vi "MQTT Session - Get TCP Info.vi"(0 "mqtt ref in":T1, 11 "error in":errorcluster) -> (4 "mqtt ref out":T1, 6 "TCP ref":refnum<k5>, 8 "TCP Timeout (ms)":i32, 10 "Version":u8, 15 "error out":errorcluster)   [LabVIEW 2019, in "KoRE-MQTT.lvlib"]
doc: "Copyright (c) 2025 KoRElibs.com\nSPDX-License-Identifier: EUPL-1.2\n\nThis VI is licensed under the European Union Public License (EUPL) Version 1.2. You may use this VI unmodified in proprietary works. If you distribute a modified version of this file, the modified file must be released under the EUPL-1.2. Full license: https://joinup.ec.europa.eu/asset/eupl/eupl/1.2/"
uses:
  KoRE-MQTT.lvlib
  Public/TypeDefs/MQTT Client Session.ctl
  TypeDefs/MQTT Client Session - Data Value Reference.ctl
  Public/TypeDefs/MQTT Client Session - Data.ctl
  Public/TypeDefs/MQTT Property - Will.ctl
  Public/TypeDefs/MQTT Property - CONNECT.ctl
  TypeDefs/MQTT Subscription - Info.ctl
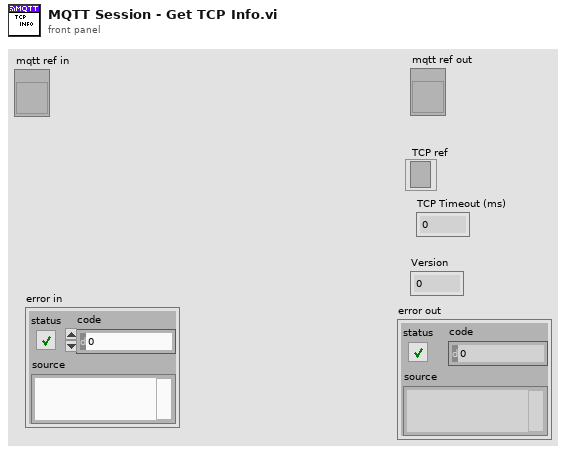
[diagram p1: front panel]
types:
  T1 = typedef "KoRE-MQTT.lvlib/MQTT Client Session.ctl" = refnum<vi>
  T2 = typedef "KoRE-MQTT.lvlib/MQTT Client Session - Data Value Reference.ctl" = refnum<data-value>
  T3 = typedef "KoRE-MQTT.lvlib/MQTT Client Session - Data.ctl" = cluster{"TCP ref":refnum<k5>, "Next Packet Id":u16, "Version":u8, "Host":string, "Port":u16, "Ping Delta":u32, "Username":string, "Password":string, "Will QoS":u8, "Will Retain":bool, "Will Topic":string, "Will Payload":string, "TCP Timeout":i32, "Semaphore":T4, "In-Flight Messages":variant, "Close":bool, "Last Send":u32, "Keep Alive":u16, "Last Ping RTT":u32, "Last Ping":u32, "Will Properties":T5[], "Session Expiry Interval":u32, "Maximum QoS":u8, "Retain Available":bool, "Server Maximum Packet Size":u32, "Client Identifier":string, "Server Topic Alias Maximum":u16, "Wildcard Subscription Available":bool, "Subscription Identifier Available":bool, "Shared Subscription Available":bool, "Connect Properties":T6[], "Client Maximum Packet Size":u32, "Client Topic Alias Maximum":u16, "Server Receive Maximum":u16, "Client Receive Maximum":u16, "TLS cfg":refnum<k36>, "Subscriptions":T7[]}
  T4 = typedef "Semaphore RefNum" = refnum<k1>
  T5 = typedef "KoRE-MQTT.lvlib/MQTT Property - Will.ctl" = cluster{"Property":u8, "Value":string}
  T6 = typedef "KoRE-MQTT.lvlib/MQTT Property - CONNECT.ctl" = cluster{"Property":u8, "Value":string}
  T7 = typedef "KoRE-MQTT.lvlib/MQTT Subscription - Info.ctl" = cluster{"Packet Id":u16, "Index":u16, "Identifier":u32, "QoS":u8, "Topic Filter":string, "Reason Code":u8, "Reason String":string, "Granted":bool}
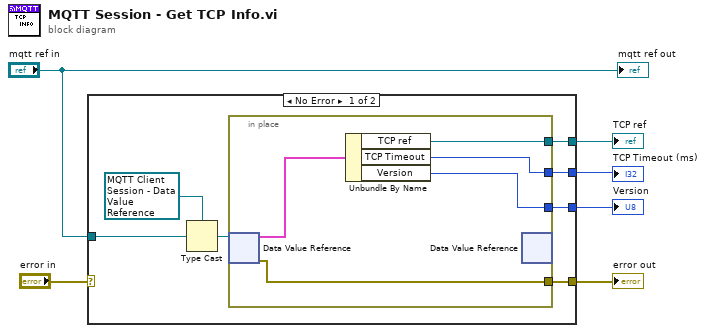
[diagram p0: block diagram]
diagram:
  n1 = case shown="No Error" "error in" {
    selector: "error in" -> [_ w19]
    tunnel: "mqtt ref in" -> [w12 _]
    tunnel: [w10 w19] -> w2
    tunnel: [w9 _] -> w4
    tunnel: [w8 _] -> w3
    tunnel: [w7 _] -> w1
    frame No Error {
      n2 = Type Cast(type=T2 refnum ("data value reference"), x=w12) -> (*(type *) &x=w11:T2)
      n3 = in-place {
        in-place-border: [w17] -> w9
        in-place-border: [w16] -> w10
        in-place-border: [w15] -> w8
        in-place-border: [w14] -> w7
        n4 = in-place-dvr #1(w11) -> (w18:T3, w16:errorcluster)
        n5 = Unbundle By Name(w18) -> ("TCP ref"=w17:refnum<k5>, "TCP Timeout"=w15:i32, "Version"=w14:u8)
        n6 = in-place-dvr #1() -> ()  [unwired: 1 in, 2 out]
      }
    }
    frame Error {
    }
  }
  "TCP ref" <- w4
  "TCP Timeout (ms)" <- w3
  "error out" <- w2
  "Version" <- w1
  "mqtt ref out" <- "mqtt ref in"
